vi "Check Order.vi"(5 "owned":i32, 6 "wallet":dbl, 7 "total":dbl, 8 "known?":bool, 9 "sell?":bool, 10 "quantity":i32, 11 "stock name":string) -> (3 "refusal":string)   [LabVIEW 2020, in "Full Featured MCP Server.lvlib"]
doc: "Checks an order before it is carried out. refusal is empty for an order that is fine; otherwise it says why the order is refused, in words the assistant can act on."
uses:
  Full Featured MCP Server.lvlib
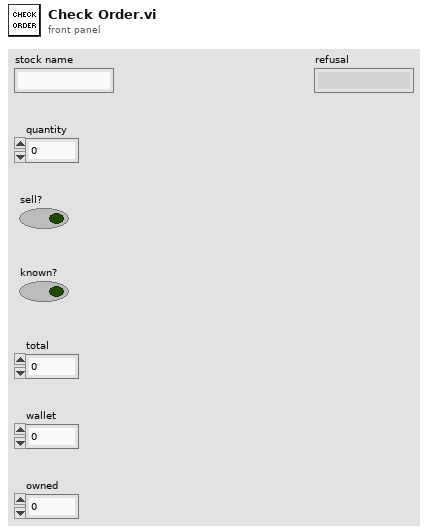
[diagram p1: front panel]
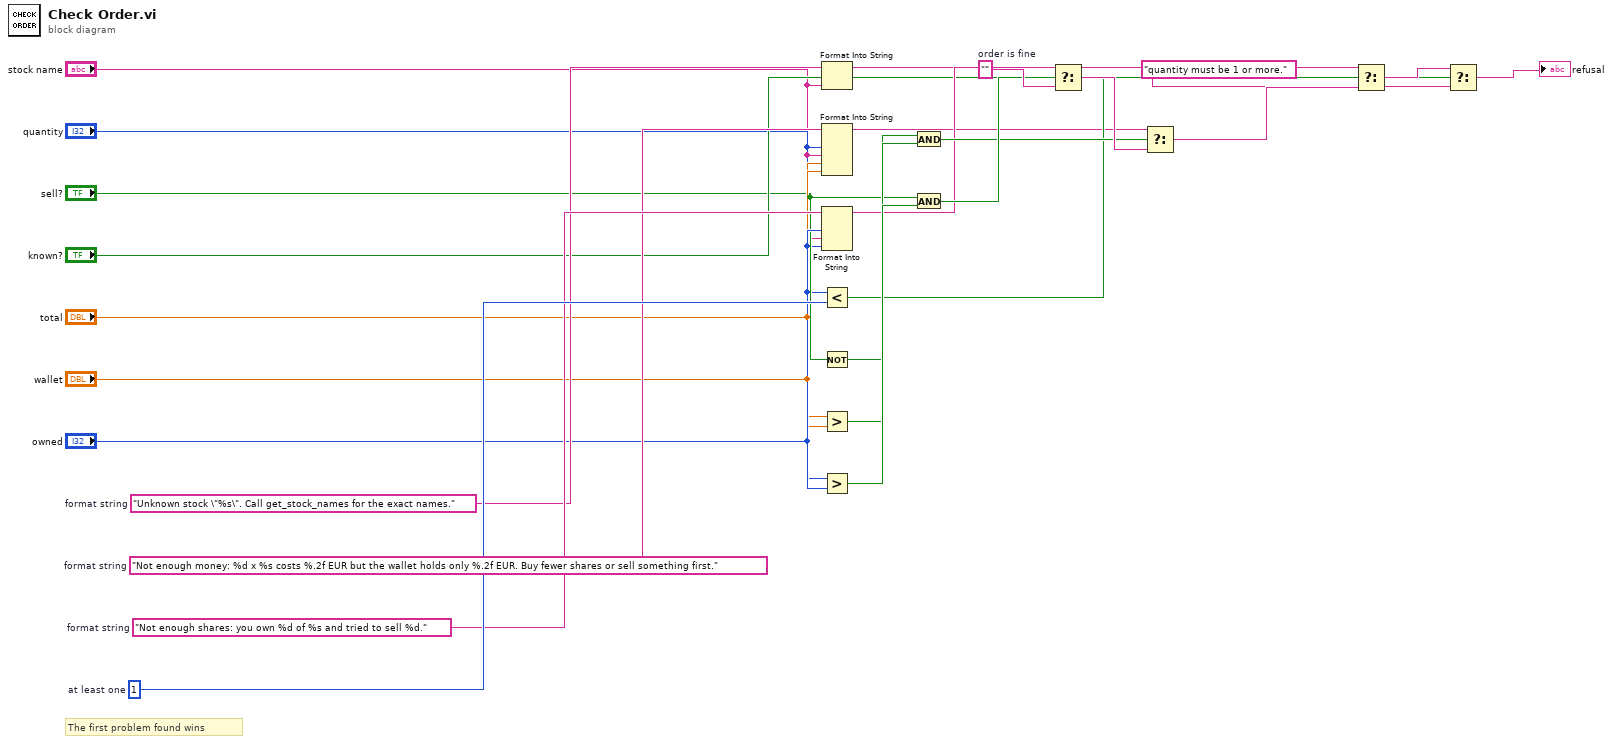
[diagram p0: block diagram]
diagram:
  w22 = ""  # order is fine
  w15 = 1  # at least one
  w13 = "Not enough shares: you own %d of %s and tried to sell %d."  # format string
  w11 = "Not enough money: %d x %s costs %.2f EUR but the wallet holds only %.2f EUR. Buy fewer shares or sell something first."  # format string
  w8 = "Unknown stock \"%s\". Call get_stock_names for the exact names."  # format string
  # "The first problem found wins"
  n1 = Format Into String(format string=w8, "stock name") -> (resulting string=w9:string)  [unwired: 2 in, 1 out]
  n2 = Format Into String(format string=w11, "quantity", "stock name", "total", "wallet") -> (resulting string=w12:string)  [unwired: 2 in, 1 out]
  n3 = Format Into String(format string=w13, "owned", "stock name", "quantity") -> (resulting string=w14:string)  [unwired: 2 in, 1 out]
  n4 = Less?(x="quantity", y=w15) -> (x < y?=w16:bool)
  n5 = Not(x="sell?") -> (.not. x?=w17:bool)
  n6 = Greater?(x="total", y="wallet") -> (0:w18:bool)
  n7 = Greater?(x="quantity", y="owned") -> (0:w20:bool)
  n8 = And(x=w17, y=w18) -> (x .and. y?=w19:bool)
  n9 = And(x="sell?", y=w20) -> (x .and. y?=w21:bool)
  n10 = Select(t=w14, s=w21, f=w22) -> (s? t:f=w23:string)
  n11 = Select(t=w12, s=w19, f=w23) -> (s? t:f=w24:string)
  n12 = Select(t="quantity must be 1 or more.", s=w16, f=w24) -> (s? t:f=w25:string)
  n13 = Select(t=w25, s="known?", f=w9) -> (s? t:f=→"refusal":string)
